vi "TC01.vi"() -> ()   [LabVIEW 2026]
uses:
  <vilib>/Utility/file.llb/Write Delimited Spreadsheet (DBL).vi
panel:
  in  "file path (dialog if empty)":path
  in  "Loop":i32
  out "ACRMS, V":dbl format="%#_3f"
  out "VPP, V":dbl format="%#_3f"
  in  "?":u32
  out "error out":errorcluster {"code" format="%f"}
  in  "DHO804":refnum<visa-resource-name>
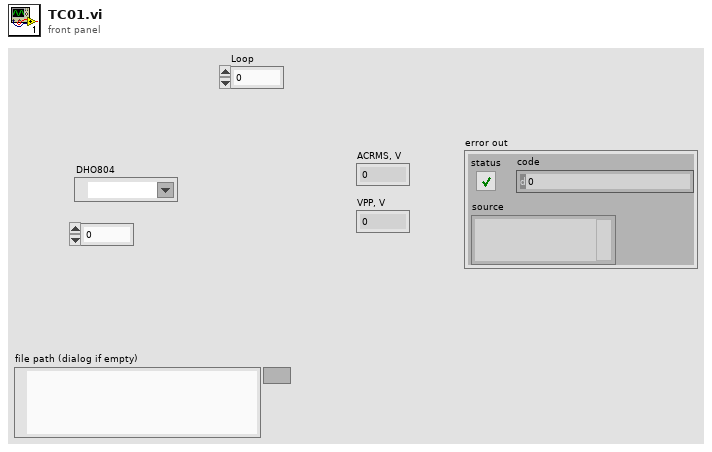
[diagram p1: front panel]
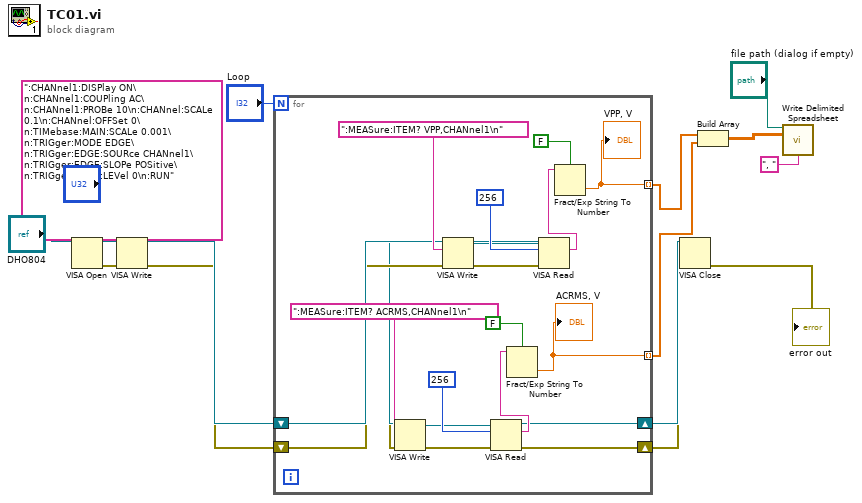
[diagram p0: block diagram]
diagram:
  n1 = VISA Open(timeout (0)="?", VISA resource name="DHO804") -> (VISA resource name=w12:refnum<visa-resource-name>, error out=w13:errorcluster)  [unwired: 3 in]
  n2 = VISA Write(VISA resource name=w12, write buffer=":CHANnel1:DISPlay ON\n:CHANnel1:COUPling AC\n:CHANnel1:PROBe 10\n:CHANnel:SCALe 0.1\n:CHANnel:OFFSet 0\n:TIMebase:MAIN:SCALe 0.001\n:TRIGger:MODE EDGE\n:TRIGger:EDGE:SOURce CHANnel1\n:TRIGger:EDGE:SLOPe POSitive\n:TRIGger:EDGE:LEVel 0\n:RUN", error in (no error)=w13) -> (VISA resource name out=w11:refnum<visa-resource-name>, error out=w10:errorcluster)  [unwired: 1 out]
  n3 = for {
    N: "Loop" -> [_]
    shift-right: [w20] -> w8
    shift-left: w11 -> [w34]
    shift-right: [w19] -> w7
    shift-left: w10 -> [w33]
    tunnel: [w18] -> w5 mode=indexing
    tunnel: [w17] -> w3 mode=indexing
    n4 = VISA Write(VISA resource name=w34, write buffer=":MEASure:ITEM? VPP,CHANnel1\n", error in (no error)=w33) -> (VISA resource name out=w32:refnum<visa-resource-name>, error out=w31:errorcluster)  [unwired: 1 out]
    n5 = VISA Read(VISA resource name=w32, byte count=u32 256, error in (no error)=w31) -> (VISA resource name out=w22:refnum<visa-resource-name>, read buffer=w30:string, error out=w21:errorcluster)  [unwired: 1 out]
    n6 = VISA Write(VISA resource name=w22, write buffer=":MEASure:ITEM? ACRMS,CHANnel1\n", error in (no error)=w21) -> (VISA resource name out=w26:refnum<visa-resource-name>, error out=w25:errorcluster)  [unwired: 1 out]
    n7 = VISA Read(VISA resource name=w26, byte count=u32 256, error in (no error)=w25) -> (VISA resource name out=w20:refnum<visa-resource-name>, read buffer=w24:string, error out=w19:errorcluster)  [unwired: 1 out]
    n8 = Fract/Exp String To Number(use system decimal point (T)=FALSE, string=w24) -> (number=w17:dbl)  [unwired: 2 in, 1 out]
    "ACRMS, V" <- w17
    n9 = Fract/Exp String To Number(use system decimal point (T)=FALSE, string=w30) -> (number=w18:dbl)  [unwired: 2 in, 1 out]
    "VPP, V" <- w18
  }
  n10 = VISA Close(VISA resource name=w8, error in (no error)=w7) -> (error out=→"error out":errorcluster)
  n11 = Build Array(w5, w3) -> (w4:dbl[][])
  n12 = call-poly <vilib>:"Write Delimited Spreadsheet.vi"("file path (dialog if empty)"="file path (dialog if empty)", "2D data"=w4, "delimiter (\\t)"=", " ("delimiter (\\t)")) -> ()  [unwired: 11 in, 2 out]
